vi "KYFG Get Camera Value Type.vi"(8 "error in (no error)":errorcluster, 10 "paramName":string, 11 "camHandle":u32) -> (0 "error out":errorcluster, 3 "function return":u32(ring))   [LabVIEW 2023, in "KYFGLib_lv.lvlib"]
doc: "KYFG_API KY_CAM_PROPERTY_TYPE KYFG_GetCameraValueType(CAMHANDLE camHandle, const char *paramName);"
uses:
  KYFGLib_lv.lvlib
  KYFGLib.dll
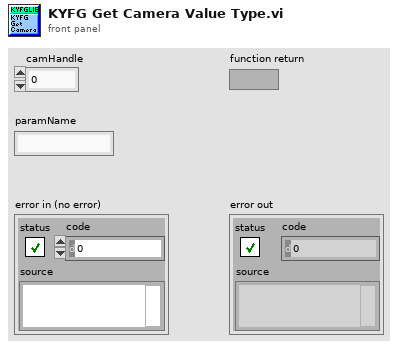
[diagram p1: front panel]
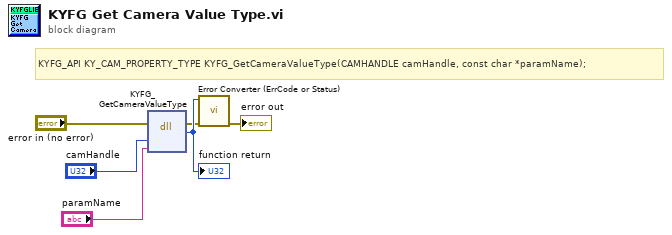
[diagram p0: block diagram]
diagram:
  # "KYFG_API KY_CAM_PROPERTY_TYPE KYFG_GetCameraValueType(CAMHANDLE camHandle, const char *paramName);"
  n1 = dll-call lib="KYFGLib.dll" fn="KYFG_GetCameraValueType"(error in="error in (no error)", "camHandle"="camHandle", "paramName"="paramName") -> (error out=w2:errorcluster, "return type"=w6:u32)  [unwired: 4 in, 1 out]
  "function return" <- w6
  n2 = call "Error Converter (ErrCode or Status).vi"("error in (no error)"=w2, "error code"=w6) -> ("error out"=→"error out":errorcluster)  [unwired: 9 in]
